vi "uRedFPGA.vi"() -> ()   [LabVIEW 2019]
uses:
  <vilib>/rvi/Emulation/niFpgaGetClockAttributes.vi
  <vilib>/rvi/Emulation/niFpgaSctlEmulationGetInTimedLoop.vi
  <vilib>/rvi/Emulation/niFpgaEmulationReportErrorSimple.vi
  <vilib>/rvi/eio/common/nirviEmuTemplateMethod_errors.vi
  <vilib>/rvi/Emulation/niFpgaCriticalErrorInLSC.vi
  <vilib>/rvi/FXPMathLib/FxpMul/XNode/nifxpmath_Multiplier.xnode
  <vilib>/rvi/FXPMathLib/FxpSub/XNode/nifxpmath_Sub.xnode
  <vilib>/eio/EIONode/EIONode.xnode
  <vilib>/rvi/FXPMathLib/sim/FxpSim.dll
panel:
  in  "Time_ms":u32=1000
  in  "LimSoC":fxp<+/-,32,16>
  out "SoCMin":bool
  out "BlocIb":bool
  out "Ib_Out":i16
  in  "1/nc(b)":fxp<+,18,2>
  in  "T/(n(CD)*Q)":fxp<+,32,2>
  in  "Q":fxp<+/-,32,16> format="%#_26g"
  in  "P*f/i_stc":fxp<+,16,0>=0.375 format="%#_16g"
  out "PL>PPV":bool
  out "Vg":bool
  out "SoC<0.8":bool
  in  "Cargar":bool
  in  "CC_Constant":fxp<+,16,0>
  out "mSoC":fxp<+/-,64,4>
  in  "P_SoC":bool
  in  "nc(b)":fxp<+,18,2>
  in  "N_Panel":fxp<+,4,4>
  out "ib":fxp<+/-,64,33>
  in  "1/Voc":fxp<+,16,8>
  out "SoC":fxp<+,32,0>
  out "PPV":fxp<+,45,21>
  out "PG":fxp<+/-,47,23>
  in  "VG":fxp<+,16,8>
  out "Pb":fxp<+/-,47,23>
  in  "T*n(CD)/Q":fxp<+,32,2>
  in  "SoC_in":fxp<+,32,0>
  in  "PL":fxp<+,45,21>
  out "Time(ms)":u32
  in  "n(p)":fxp<+,16,0>
  in  "G":fxp<+,16,14>
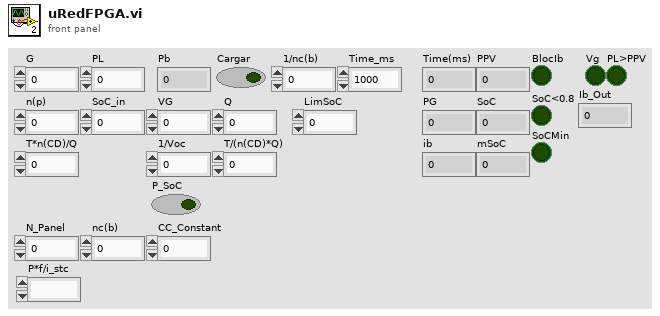
[diagram p1: front panel]
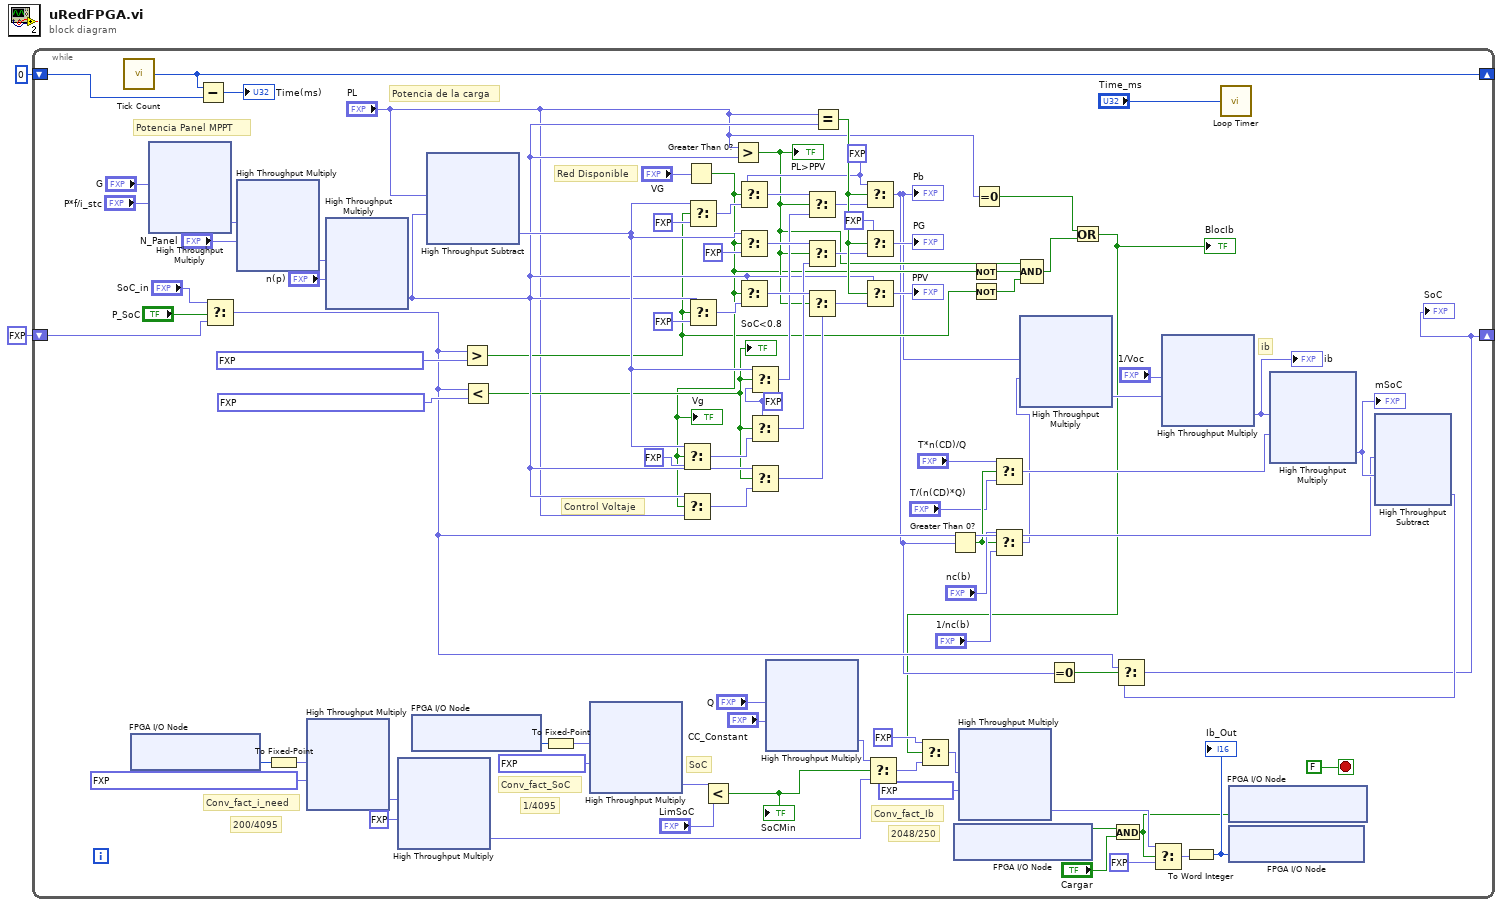
[diagram p0: block diagram]
diagram:
  n1 = while {
    shift-right: [w93] -> _
    shift-left: u32 0 ("Tick Count(Ticks)") -> [w92]
    shift-right: [w65] -> _
    shift-left: fxp<+,32,0> 0.0 ("x-y") -> [w61]
    stop <- FALSE stop-if-true
    w29 = fxp<+,45,21> 0.0 ("t")
    w31 = fxp<+,45,21> 0.0 ("t")
    # "200/4095"
    # "Conv_fact_i_need"
    # "2048/250"
    # "1/4095"
    # "Conv_fact_Ib"
    # "SoC"
    # "Conv_fact_SoC"
    # "Control Voltaje"
    # "Red Disponible"
    # "ib"
    # "Potencia de la carga"
    # "Potencia Panel MPPT"
    n2 = call "Tick Count"() -> ("Tick Count(mSec)"=w93:u32)
    n3 = xnode "FPGA I/O Node"() -> ("ConnectorA/AI1"=w42:u16)  [unwired: 1 in, 1 out]
    n4 = xnode ("High Throughput Multiply")("x"="G", "y"="P*f/i_stc") -> ("x*y"=w33:fxp<+,32,14>)
    n5 = Subtract(x=w93, y=w92) -> (x-y=→"Time(ms)":u32)
    n6 = Select(t="SoC_in", s="P_SoC", f=w61) -> (s? t:f=w60:fxp<+,32,0>)
    n7 = xnode ("High Throughput Multiply")("x"=w33, "y"="N_Panel") -> ("x*y"=w58:fxp<+,36,18>)
    n8 = To Fixed-Point(number=w42) -> (fixed-point=w41:fxp<+,16,16>)  [unwired: 1 in]
    n9 = xnode ("High Throughput Multiply")("x"=w41, "y"=fxp<+,32,0> 0.04884000006131828) -> ("x*y"=w39:fxp<+,48,16>)
    n10 = xnode ("High Throughput Multiply")("x"=w58, "y"="n(p)") -> ("x*y"=w57:fxp<+,45,21>)
    n11 = xnode ("High Throughput Multiply")("x"=w39, "y"=fxp<+/-,1,1> -1.0) -> ("x*y"=w37:fxp<+/-,32,16>)
    n12 = xnode "FPGA I/O Node"() -> ("ConnectorA/AI0"=w54:u16)  [unwired: 1 in, 1 out]
    n13 = xnode "High Throughput Subtract"("x"="PL", "y"=w57) -> ("x-y"=w71:fxp<+/-,47,23>)
    n14 = Greater?(x=w60, y=fxp<+,32,0> 0.30000000004656613) -> (0:w22:bool)
    n15 = Less?(x=w60, y=fxp<+,32,0> 0.8000000000465661) -> (x < y?=w34:bool)
    "SoC<0.8" <- w34
    n16 = To Fixed-Point(number=w54) -> (fixed-point=w53:fxp<+,16,16>)  [unwired: 1 in]
    n17 = xnode ("High Throughput Multiply")("x"=w53, "y"=fxp<+/-,16,0> 0.000244140625) -> ("x*y"=w51:fxp<+/-,32,16>)
    n18 = Greater Than 0?(x="VG") -> (x > 0?=w23:bool)
    "Vg" <- w23
    n19 = Select(t=w71, s=w23, f=fxp<+,45,21> 0.0 ("t")) -> (s? t:f=w73:fxp<+/-,47,23>)
    n20 = Select(t=w57, s=w23, f="PL") -> (s? t:f=w72:fxp<+,45,21>)
    n21 = Select(t=w71, s=w22, f=fxp<+/-,45,21> 0.0) -> (s? t:f=w79:fxp<+/-,47,23>)
    n22 = Select(t=w57, s=w22, f=fxp<+,45,21> 0.0) -> (s? t:f=w78:fxp<+,45,21>)
    n23 = Less?(x=w51, y="LimSoC") -> (x < y?=w6:bool)
    "SoCMin" <- w6
    n24 = Greater?(x="PL", y=w57) -> (0:w26:bool)
    "PL>PPV" <- w26
    n25 = Select(t=w31, s=w23, f=w79) -> (s? t:f=w82:fxp<+/-,47,23>)
    n26 = Select(t=w71, s=w23, f=fxp<+,45,21> 0.0 ("t")) -> (s? t:f=w81:fxp<+/-,47,23>)
    n27 = Select(t=w57, s=w23, f=w78) -> (s? t:f=w80:fxp<+,45,21>)
    n28 = Select(t=w71, s=w34, f=w29) -> (s? t:f=w76:fxp<+/-,47,23>)
    n29 = Select(t=w29, s=w34, f=w73) -> (s? t:f=w75:fxp<+/-,47,23>)
    n30 = Select(t=w57, s=w34, f=w72) -> (s? t:f=w74:fxp<+,45,21>)
    n31 = xnode ("High Throughput Multiply")("x"="Q", "y"="CC_Constant") -> ("x*y"=w36:fxp<+/-,32,16>)
    n32 = Select(t=w82, s=w26, f=w76) -> (s? t:f=w85:fxp<+/-,47,23>)
    n33 = Select(t=w81, s=w26, f=w75) -> (s? t:f=w84:fxp<+/-,47,23>)
    n34 = Select(t=w80, s=w26, f=w74) -> (s? t:f=w83:fxp<+,45,21>)
    n35 = Equal?(x="PL", y=w57) -> (x = y?=w87:bool)
    n36 = Select(t=w31, s=w87, f=w85) -> (s? t:f=w9:fxp<+/-,47,23>)
    "Pb" <- w9
    n37 = Select(t=fxp<+,45,21> 0.0, s=w87, f=w84) -> (s? t:f=→"PG":fxp<+/-,47,23>)
    n38 = Select(t=w57, s=w87, f=w83) -> (s? t:f=→"PPV":fxp<+,45,21>)
    n39 = Select(t=w36, s=w6, f=w37) -> (s? t:f=w21:fxp<+/-,32,16>)
    n40 = Greater Than 0?(x=w9) -> (x > 0?=w13:bool)
    n41 = xnode "FPGA I/O Node"() -> ("ConnectorC/DIO7"=w49:bool)  [unwired: 1 in, 1 out]
    n42 = Not(x=w23) -> (.not. x?=w25:bool)
    n43 = Not(x=w22) -> (.not. x?=w24:bool)
    n44 = Equal To 0?(x="PL") -> (x = 0?=w16:bool)
    n45 = Select(t="T*n(CD)/Q", s=w13, f="T/(n(CD)*Q)") -> (s? t:f=w10:fxp<+,32,2>)
    n46 = Select(t="nc(b)", s=w13, f="1/nc(b)") -> (s? t:f=w7:fxp<+,18,2>)
    n47 = xnode ("High Throughput Multiply")("x"=w9, "y"=w7) -> ("x*y"=w55:fxp<+/-,64,25>)
    n48 = Compound Arithmetic op=AND(w26, w25, w24) -> (w18:bool)
    n49 = Equal To 0?(x=w9) -> (x = 0?=w67:bool)
    n50 = Or(x=w16, y=w18) -> (x .or. y?=w4:bool)
    "BlocIb" <- w4
    n51 = Select(t=fxp<+/-,32,16> 0.0 ("f"), s=w4, f=w21) -> (s? t:f=w27:fxp<+/-,32,16>)
    n52 = xnode ("High Throughput Multiply")("x"=w27, "y"=fxp<+,16,6> 8.1923828125) -> ("x*y"=w47:fxp<+/-,48,15>)
    n53 = And(x=w49, y="Cargar") -> (x .and. y?=w43:bool)
    n54 = Select(t=w47, s=w43, f=fxp<+/-,48,15> 0.0) -> (s? t:f=w45:fxp<+/-,48,15>)
    n55 = xnode ("High Throughput Multiply")("x"="1/Voc", "y"=w55) -> ("x*y"=w8:fxp<+/-,64,33>)
    "ib" <- w8
    n56 = To Word Integer(number=w45) -> (16bit integer=w44:i16)
    "Ib_Out" <- w44
    n57 = call "Loop Timer"("Count(mSec)"="Time_ms") -> ()  [unwired: 1 out]
    n58 = xnode "FPGA I/O Node"("ConnectorC/DIO6"=w43) -> ()  [unwired: 1 in, 1 out]
    n59 = xnode "FPGA I/O Node"("ConnectorC/AO0"=w44) -> ()  [unwired: 1 in, 1 out]
    n60 = xnode ("High Throughput Multiply")("x"=w8, "y"=w10) -> ("x*y"=w90:fxp<+/-,64,4>)
    "mSoC" <- w90
    n61 = xnode "High Throughput Subtract"("x"=w60, "y"=w90) -> ("x-y"=w66:fxp<+,32,0>)
    n62 = Select(t=w60, s=w67, f=w66) -> (s? t:f=w65:fxp<+,32,0>)
    "SoC" <- w65
  }
